vi "[ex ce] Simple Sound Application.vi"() -> ()   [LabVIEW 2021]
doc: "This example demonstrates how you can perform data acqusition, processing and output from within a CalcExpress script. For the basis, simple sound application is taken.\n\nTo perform data acquisition and output, example scripts use <B>user-defined</B> functions implemented as VIs (FuncVI mechanism). <B>SndIn</B> function is used to read data from a sound input device. <B>SndOut</B> function is used to play sound on a sound output device. FuncVIs of these functions are located in <B>SndFuncVIs.llb</B>.\n\nYou need the <B>LabVIEW Advanced Analysis VIs</B> to run some scripts in this example VI.\n\n::: CalcExpress Toolkit :::\nCopyright (c) 2000-2026 Konstantin Shifershteyn. All rights reserved."
panel:
  out "in work":bool
  in  "exec":bool
  in  "sel":u16(ring) items=["***  Click here to select an example script  ***", "Script 1. Simple Data Acquisition", "Script 2. Data Acquisition and Spectrum Computing", "Script 3. Data Acquisition, Filtration and Spectrum Computing", "Script 4. Data Acquisition, Signal Processing and Playing", "Script 5. Signal Generation"]
  in  "stop":bool
  out "graph":dbl[](graph)
  in  "variable to plot":string="data"
  in  "script":string="/*\nStart this VI and select an example script in the ring above for placing it into this text box.\n\nClick Exec button to process a script.\n*/\n"
  # "NOTE. Some functions in this example use Advanced Analysis VIs.\nThe example doesn't work properly if you don't have these VIs."
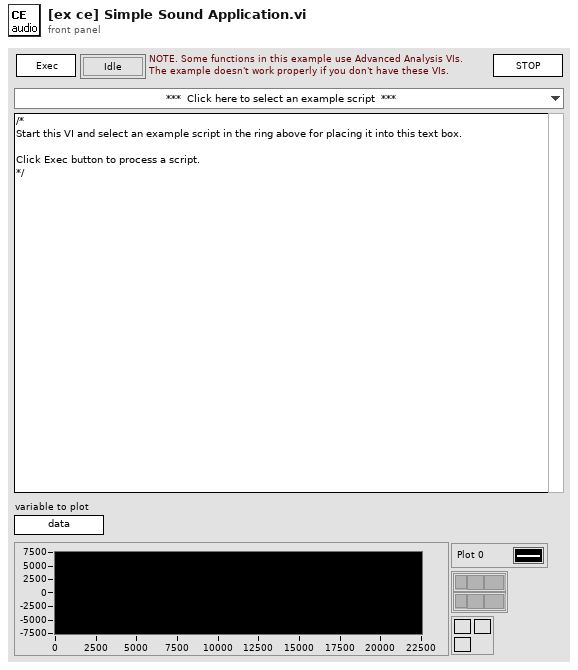
[diagram p1: front panel]
types:
  T1 = typedef "VarMan Variable Context Handle.ctl" = i32
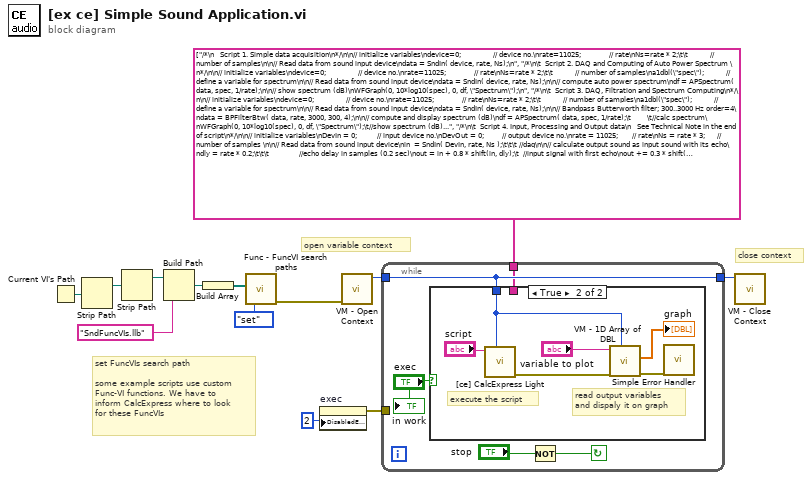
[diagram p0: block diagram]
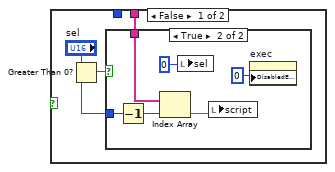
[diagram p2: hidden frame]
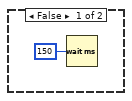
[diagram p3: hidden frame]
diagram:
  # "close context"
  # "open variable context"
  # "set FuncVIs search path\n\nsome example scripts use custom\nFunc-VI functions. We have to\ninform CalcExpress where to look\nfor these FuncVIs"
  n1 = Current VI's Path() -> (path=w10:path)
  n2 = Strip Path(path=w10) -> (stripped path=w7:path)  [unwired: 1 out]
  n3 = Strip Path(path=w7) -> (stripped path=w6:path)  [unwired: 1 out]
  n4 = Build Path(base path=w6, name or relative path="SndFuncVIs.llb") -> (appended path=w4:path)
  n5 = Build Array(w4) -> (w9:path[])
  n6 = call "Func - FuncVI search paths.vi"("cmd"=enum16{"get", "set"}."set", "user paths"=w9) -> ("error out"=w3:errorcluster)  [unwired: 4 in, 3 out]
  n7 = property on="exec" class="Bool"("DisabledEnum"=u8 2) -> (error out=w1:errorcluster)  [unwired: 2 in, 1 out]
  n8 = call "VM - Open Context.vi"("error in"=w3) -> ("VC Handle out"=w13:T1)  [unwired: 8 in, 2 out]
  n9 = while {
    tunnel: string[] ["/*\n   Script 1. Simple data acquisition\n*/\n\n// initialize variables\ndevice=0;                // device no.\nrate=11025;              // rate\nNs=rate * 2;\t\t           // number of samples\n\n// Read data from sound input device\ndata = SndIn( device, rate, Ns);\n", "/*\n\t  Script 2. DAQ and Computing of Auto Power Spectrum \n*/\n\n// initialize variables\ndevice=0;                // device no.\nrate=11025;              // rate\nNs=rate * 2;\t\t           // number of samples\na1dbl(\"spec\");           // define a variable for spectrum\n\n// Read data from sound input device\ndata = SndIn( device, rate, Ns);\n\n// compute auto power spectrum\ndf = APSpectrum( data, spec, 1/rate);\n\n// show spectrum (dB)\nWFGraph(0, 10*log10(spec), 0, df, \"Spectrum\");\n", "/*\n\t  Script 3. DAQ, Filtration and Spectrum Computing\n*/\n\n// initialize variables\ndevice=0;                // device no.\nrate=11025;              // rate\nNs=rate * 2;\t\t           // number of samples\na1dbl(\"spec\");           // define a variable for spectrum\n\n// Read data from sound input device\ndata = SndIn( device, rate, Ns);\n\n// Bandpass Butterworth filter; 300..3000 Hz order=4\ndata = BPFilterBtw( data, rate, 3000, 300, 4);\n\n// compute and display spectrum (dB)\ndf = APSpectrum( data, spec, 1/rate);\t        \t//calc spectrum\nWFGraph(0, 10*log10(spec), 0, df, \"Spectrum\");\t//show spectrum (dB)\n", "/*\n\t  Script 4. Input, Processing and Output data\n   See Technical Note in the end of script\n*/\n\n// initialize variables\nDevIn = 0;          // input device no.\nDevOut = 0;         // output device no.\nrate = 11025;       // rate\nNs = rate * 3;      // number of samples \n\n// Read data from sound input device\nin  = SndIn( DevIn, rate, Ns );\t\t\t //daq\n\n// calculate output sound as input sound with its echo\ndly = rate * 0.2;\t\t\t               //echo delay in samples (0.2 sec)\nout = in + 0.8 * shift(in, dly);\t  //input signal with first echo\nout += 0.3 * shift(in, dly*2);\t\t   //add second echo\n\nMsgBox(\"Click button to play\");    //message box\n\n// play resulting sound\nSndOut( DevOut, rate, out);\n\ndata = out;                        //for graph\n\n/*\n   Technical note.\nWhen you execute the script at the first time, you have an input\nsound in the variable 'in' and resulting sound in the variable 'out'.\nFor each new execution of the script you will have new values for\n'in' and 'out'. Let's assume that you want to compute various values\nof 'out' for one value of 'in' (to change computation algorithm of\n'out' for one set of input data or for multiple playing). For this\npurpose, it's enough to locate the SndIn function in the comment (or\nto delete from the script) after the necessary value of 'in' is\nobtained. After that, you can execute the script many time for one\nentry sound.\n*/\n", "/*\n   Script 5. Simple Signal Generation\n*/\n\n// initialize variables\ndevice=0;\nrate=11025;\nNs=rate*1;\na1dbl(\"data\");\na1dbl(\"shape\");\n\n// generate data for playing\nSquareWave(shape, Ns,    5/rate, 1, -90);\nshape = clip(shape);\nSineWave(data, Ns, 1000/rate, 20000, 0);\ndata *= shape;\n\n// play resulting data\nSndOut(device, rate, data);\n"] -> [w14]
    tunnel: [w15] -> w12
    tunnel: w13 -> [w15]
    tunnel: w1 -> [_]
    stop <- w16 continue-if-true
    n10 = case shown="True" "exec" {
      tunnel: w15 -> [_ w29]
      tunnel: w14 -> [w19 _]
      frame False {
        n11 = Greater Than 0?(x="sel") -> (x > 0?=w21:bool)
        n12 = case shown="True" w21 {
          tunnel: "sel" -> [_ w27]
          tunnel: w19 -> [_ w24]
          frame False {
            n13 = Wait (ms)(milliseconds to wait=u32 150) -> ()  [unwired: 1 out]
          }
          frame True {
            n14 = Decrement(x=w27) -> (x-1=w26:u16)
            n15 = Index Array(array=w24, index=w26) -> (element=w28:string)
            n16 = local write "sel"(u16 0) -> ()
            n17 = local write "script"(w28) -> ()
            n18 = property on="exec" class="Bool"("DisabledEnum"=u8 0) -> ()  [unwired: 2 in, 2 out]
          }
        }
      }
      frame True {
        # "read output variables\nand dispaly it on graph"
        # "execute the script"
        n19 = call "[ce] CalcExpress Light.vi"("VC Handle"=w29, "expression"="script") -> ("error out"=w31:errorcluster)  [unwired: 7 in, 2 out]
        n20 = call "VM - 1D Array of DBL.vi"("VC Handle"=w29, "error in"=w31, "name_spec"="variable to plot") -> ("error out"=w30:errorcluster, "value out"=→"graph":dbl[])  [unwired: 3 in, 4 out]
        n21 = call <vilib>:"Simple Error Handler.vi"("error in (no error)"=w30) -> ()  [unwired: 4 in, 5 out]
      }
    }
    n22 = Not(x="stop") -> (.not. x?=w16:bool)
    "in work" <- "exec"
  }
  n23 = call "VM - Close Context.vi"("VC Handle"=w12) -> ()  [unwired: 9 in, 2 out]
